vi "Save DAC Configuration.vi"(8 "error in":errorcluster, 10 "Config File refnum in":T1, 11 "DAC Keller BNC in":refnum<class "DAC Keller BNC.lvclass">) -> (0 "error out":errorcluster, 2 "Config File refnum out":T1, 3 "DAC Keller BNC out":refnum<class "DAC Keller BNC.lvclass">)   [LabVIEW 2019, in "DAC.lvlib" / "DAC Keller BNC.lvclass"]
uses:
  DAC Keller BNC.lvclass
  <vilib>/Utility/config.llb/Write Key (String).vi
  <vilib>/Utility/config.llb/Write Key (I32).vi
  DAC.lvclass
  <vilib>/Utility/config.llb/NI_LVConfig.lvlib
  <vilib>/Utility/config.llb/Config Data RefNum.ctl
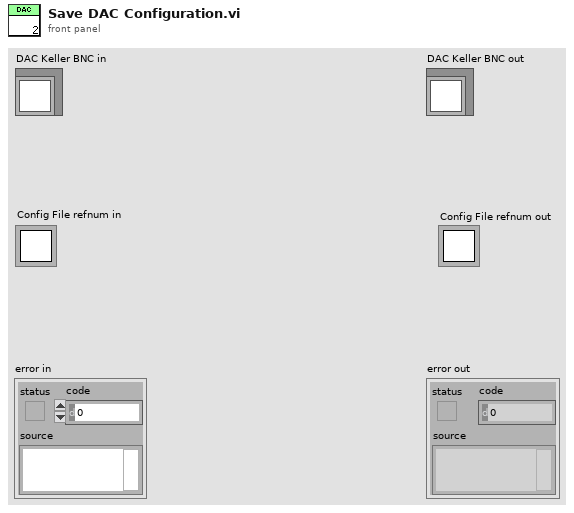
[diagram p1: front panel]
types:
  T1 = typedef "NI_LVConfig.lvlib/Config Data RefNum.ctl" = refnum<k1>
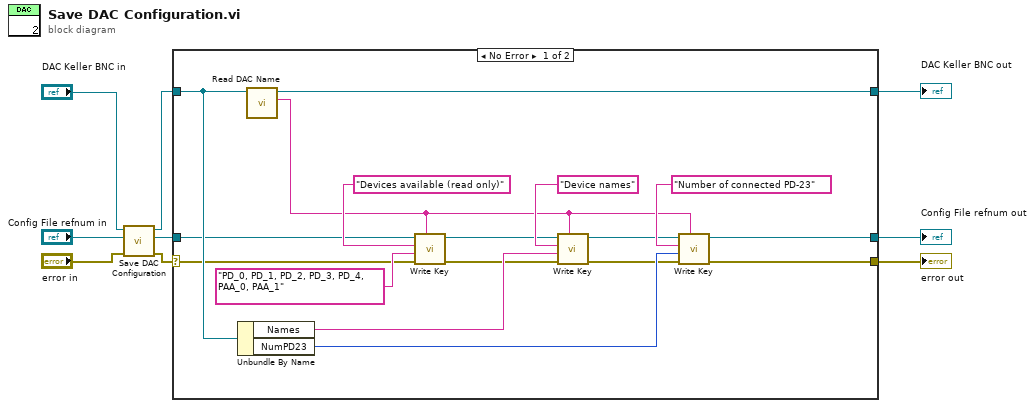
[diagram p0: block diagram]
diagram:
  n1 = call-parent "Save DAC Configuration.vi"("error in"="error in", "Config File refnum in"="Config File refnum in", "DAC in"="DAC Keller BNC in") -> ("error out"=w4:errorcluster, "Config File refnum out"=w5:T1, "DAC out"=w6:refnum<class "DAC Keller BNC.lvclass">)  [unwired: 6 in]
  n2 = case shown="No Error" w4 {
    selector: w4 -> [w19 w29]
    tunnel: [w11 w29] -> w1
    tunnel: [w24 w28] -> w3
    tunnel: w6 -> [w25 w28]
    tunnel: w5 -> [w18 w27]
    tunnel: [w13 w27] -> w2
    frame No Error {
      n3 = Unbundle By Name(w25) -> ("Names"=w23:string, "NumPD23"=w15:i32)
      n4 = call "Read DAC Name.vi"("DAC in"=w25) -> ("DAC Name"=w10:string, "DAC out"=w24:refnum<class "DAC Keller BNC.lvclass">)  [unwired: 8 in, 1 out]
      n5 = call-poly <vilib>:"Write Key.vi"("section"=w10, "error in (no error)"=w19, "value"="PD_0, PD_1, PD_2, PD_3, PD_4, PAA_0, PAA_1", "key"="Devices available (read only)", "refnum"=w18) -> ("error out"=w20:errorcluster, "refnum out"=w17:T1)  [unwired: 4 in, 1 out]
      n6 = call-poly <vilib>:"Write Key.vi"("section"=w10, "error in (no error)"=w20, "value"=w23, "key"="Device names", "refnum"=w17) -> ("error out"=w12:errorcluster, "refnum out"=w14:T1)  [unwired: 4 in, 1 out]
      n7 = call-poly <vilib>:"Write Key.vi"("section"=w10, "error in (no error)"=w12, "value"=w15, "key"="Number of connected PD-23", "refnum"=w14) -> ("error out"=w11:errorcluster, "refnum out"=w13:T1)  [unwired: 4 in, 1 out]
    }
    frame Error {
    }
  }
  "error out" <- w1
  "DAC Keller BNC out" <- w3
  "Config File refnum out" <- w2
